vi "Module Init.vi"(8 "error in (no error)":errorcluster, 11 "ValveSimModule in":refnum<class "ValveSimModule.lvclass">) -> (0 "error out":errorcluster, 3 "ValveSimModule out":refnum<class "ValveSimModule.lvclass">)   [LabVIEW 2020, in "VolatusScratch.lvlib" / "ValveSimModule.lvclass"]
uses:
  ValveSimModule.lvclass
  ValveSimModule.lvclass/ValveSimModule.ctl
  Volatus/Module/Module.lvclass
  VolatusConfig/Task/Task Config.lvclass
  VolatusConfig/VolatusConfigElement/VolatusConfigElement.lvclass
  C:/dev/lv20CE/relink/lv-volatus/Volatus/Module/Module.lvclass
  C:/dev/lv20CE/relink/lv-volatus/VolatusScratch/ValveSimModule/ValveSimModule.lvclass
  lv-vecto/Vecto/Group DBL/Group DBL.lvclass
  Volatus/Message Registration.ctl
  Volatus/Volatus.lvlib
  C:/dev/lv20CE/relink/lv-vecto/Vecto/Group/Group.lvclass
  C:/dev/lv20CE/relink/lv-vecto/Vecto/Group DBL/Group DBL.lvclass
  VolatusConfig/Group/Group Config.lvclass
  C:/dev/lv20CE/relink/lv-volatus/VolatusConfig/VolatusConfigElement/VolatusConfigElement.lvclass
  C:/dev/lv20CE/relink/lv-volatus/VolatusConfig/Group/Group Config.lvclass
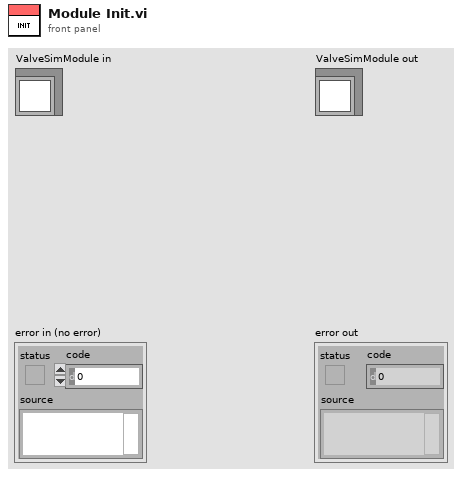
[diagram p1: front panel]
types:
  T1 = typedef "Volatus.lvlib/Message Registration.ctl" = cluster{"Message Type":string, "Message ID":string}
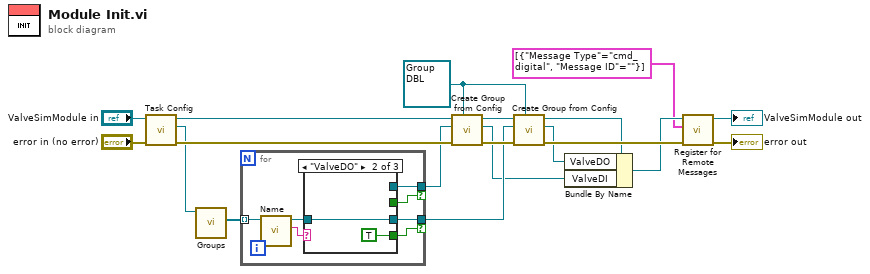
[diagram p0: block diagram]
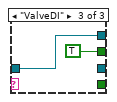
[diagram p3: hidden frame]
diagram:
  w9 = refnum<class "Group DBL.lvclass"> refnum ("ValveDI")
  n1 = call "Task Config.vi"("error in (no error)"="error in (no error)", "Module in"="ValveSimModule in") -> ("error out"=w17:errorcluster, "Task Config"=w16:refnum<class "Task Config.lvclass">, "Module out"=w13:refnum<class "ValveSimModule.lvclass">)  [unwired: 7 in]
  n2 = call "Groups.vi"("Task in"=w16) -> ("Groups"=w15:refnum<class "Group Config.lvclass">[])  [unwired: 8 in, 2 out]
  n3 = for {
    tunnel: w15 -> [w26] mode=indexing
    tunnel: [w23] -> w8 if=w22
    tunnel: [w21] -> w12 if=w20
    n4 = call "Name.vi"("VolatusConfigElement in"=w26) -> ("Name"=w25:string, "VolatusConfigElement out"=w24:refnum<class "Group Config.lvclass">)  [unwired: 8 in, 1 out]
    n5 = case shown="\"ValveDO\"" w25 {
      tunnel: w24 -> [_ w28 w30]
      tunnel: [_ w28 _] -> w23
      tunnel: [_ TRUE _] -> w22
      tunnel: [_ _ w30] -> w21
      tunnel: [_ _ TRUE] -> w20
      frame Default {
      }
      frame "ValveDO" {
      }
      frame "ValveDI" {
      }
    }
  }
  n6 = call "Create Group from Config.vi"("Group Type (Abstract)"=w9, "error in (no error)"=w17, "Group Config"=w12, "Module in"=w13) -> ("error out"=w14:errorcluster, "Group"=w6:refnum<class "Group DBL.lvclass">, "Module out"=w10:refnum<class "ValveSimModule.lvclass">)  [unwired: 5 in]
  n7 = call "Create Group from Config.vi"("Group Type (Abstract)"=w9, "error in (no error)"=w14, "Group Config"=w8, "Module in"=w10) -> ("error out"=w11:errorcluster, "Group"=w7:refnum<class "Group DBL.lvclass">, "Module out"=w5:refnum<class "ValveSimModule.lvclass">)  [unwired: 5 in]
  n8 = Bundle By Name(cluster=w5, "ValveDO"=w7, "ValveDI"=w6) -> (w4:refnum<class "ValveSimModule.lvclass">)
  n9 = call "Register for Remote Messages.vi"("error in (no error)"=w11, "Messages"=T1[] [{"Message Type"="cmd_digital", "Message ID"=""}], "Module in"=w4) -> ("error out"=→"error out":errorcluster, "Module out"=→"ValveSimModule out":refnum<class "ValveSimModule.lvclass">)  [unwired: 7 in]
